vi "benchmarks_largeBinarySHA1.vi"() -> ()   [LabVIEW 2013]
uses:
  SHA-1/SHA-1.lvclass
  <vilib>/Analysis/baseanly.llb/Mean (DBL).vi
  <vilib>/Analysis/NI_AALBase.lvlib
  SHA-1/SHA-1.lvlib
panel:
  out "MISSING ALGORITHM":bool
  out "equal hashes":bool
  out "% gain":dbl
  out "LVOS":dbl
  out "Other Algorithm":dbl
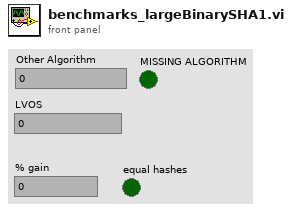
[diagram p1: front panel]
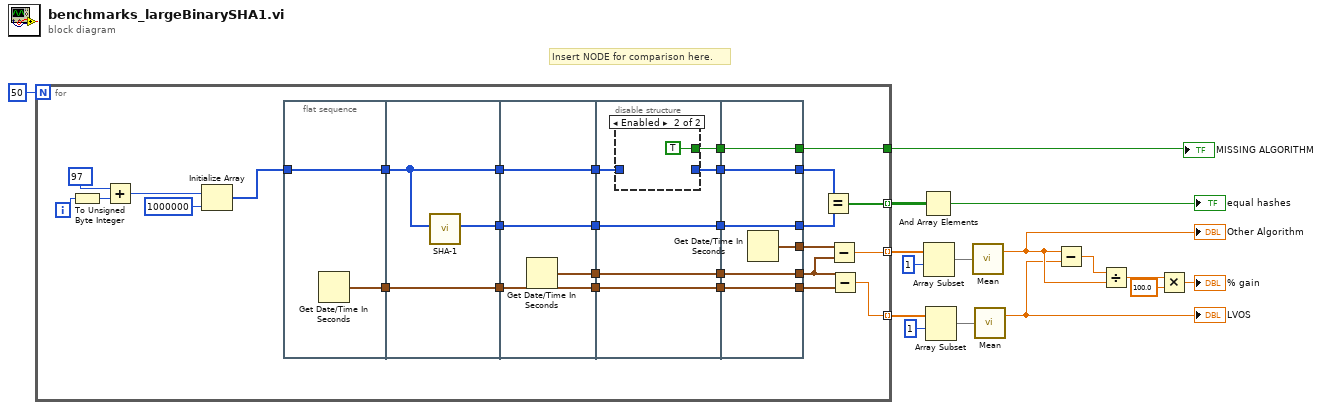
[diagram p0: block diagram]
diagram:
  # "Insert NODE for comparison here."
  n1 = for {
    N: 50 -> [_]
    tunnel: [w30] -> w16 mode=indexing
    tunnel: [w29] -> w9 mode=indexing
    tunnel: [w28] -> w8 mode=indexing
    tunnel: [w18] -> w1
    i -> [w22]
    n2 = To Unsigned Byte Integer(number=w22) -> (unsigned 8bit integer=w19:u8)
    n3 = Add(x=u8 97 ("Numeric"), y=w19) -> (x+y=w20:u8)
    n4 = Initialize Array(w20, 1000000 ("dimension size")) -> (w23:u8[])
    n5 = flat-sequence {
      tunnel: w23 -> [w47]
      tunnel: [w47] -> w45
      tunnel: [w46] -> w44
      tunnel: [w49] -> w43
      tunnel: w45 -> [w49]
      tunnel: w44 -> [w50]
      tunnel: [w50] -> w42
      tunnel: [w48] -> w27
      tunnel: w43 -> [w54]
      tunnel: [w54] -> w41
      tunnel: [w53] -> w40
      tunnel: [w52] -> w39
      tunnel: w42 -> [w52]
      tunnel: w27 -> [w51]
      tunnel: [w51] -> w26
      tunnel: w41 -> [w57]
      tunnel: [w60] -> w38
      tunnel: w40 -> [w60]
      tunnel: [w59] -> w37
      tunnel: w39 -> [w59]
      tunnel: [w56] -> w36
      tunnel: w26 -> [w58]
      tunnel: [w58] -> w25
      tunnel: [w55] -> w17
      tunnel: [w68] -> w34
      tunnel: w38 -> [w68]
      tunnel: [w67] -> w33
      tunnel: w37 -> [w67]
      tunnel: [w66] -> w35
      tunnel: [w65] -> w32
      tunnel: w36 -> [w65]
      tunnel: [w64] -> w31
      tunnel: w25 -> [w64]
      tunnel: [w63] -> w18
      tunnel: w17 -> [w63]
      frame #0 {
        n6 = Get Date/Time In Seconds() -> (seconds since 1Jan1904=w46:timestamp)
      }
      frame #1 {
        n7 = call "SHA-1.vi"("data"=w49) -> ("SHA-1 hash"=w48:u8[])  [unwired: 10 in]
      }
      frame #2 {
        n8 = Get Date/Time In Seconds() -> (seconds since 1Jan1904=w53:timestamp)
      }
      frame #3 {
        n9 = disable-structure shown="Enabled" {
          disable-tunnel: [w61 _] -> w56
          disable-tunnel: w57 -> [w61 _]
          disable-tunnel: [_ TRUE] -> w55
          frame Disabled {
          }
          frame Enabled {
          }
        }
      }
      frame #4 {
        n10 = Get Date/Time In Seconds() -> (seconds since 1Jan1904=w66:timestamp)
      }
    }
    n11 = Equal?(x=w32, y=w31) -> (x = y?=w30:bool[])
    n12 = Subtract(x=w35, y=w34) -> (x-y=w29:dbl)
    n13 = Subtract(x=w34, y=w33) -> (x-y=w28:dbl)
  }
  "MISSING ALGORITHM" <- w1
  n14 = And Array Elements(Boolean array=w16) -> (logical AND=→"equal hashes":bool)
  n15 = Array Subset(array=w9, index=1) -> (w12:dbl[])  [unwired: 1 in]
  n16 = Array Subset(array=w8, index=1) -> (w11:dbl[])  [unwired: 1 in]
  n17 = call-poly <vilib>:"Mean.vi"("X"=w12) -> ("mean"=w4:dbl)  [unwired: 1 out]
  "Other Algorithm" <- w4
  n18 = call-poly <vilib>:"Mean.vi"("X"=w11) -> ("mean"=w3:dbl)  [unwired: 1 out]
  "LVOS" <- w3
  n19 = Subtract(x=w4, y=w3) -> (x-y=w7:dbl)
  n20 = Divide(x=w7, y=w4) -> (x/y=w5:dbl)
  n21 = Multiply(x=w5, y=100.0) -> (x*y=→"% gain":dbl)
